vi "TargetArchsHasBin.vi"(8 "error in":errorcluster, 10 "MinorVersion":i32, 11 "MajorVersion":i32) -> (0 "error out":errorcluster, 3 "HasBinary":bool)   [LabVIEW 2020, in "OpenLvVision_OpenCv.lvlib" / "Cuda.lvlib"]
doc: "Check whether the module contains binary CUDA code for the given architecture"
uses:
  Cuda.lvlib
  OpenLvVision_OpenCv.lvlib
  <vilib>/Utility/error.llb/Error Cluster From Error Code.vi
  <vilib>/ErrorRing/Error Ring.xnode
  Dlls/OlvOpenCvWrapper.dll
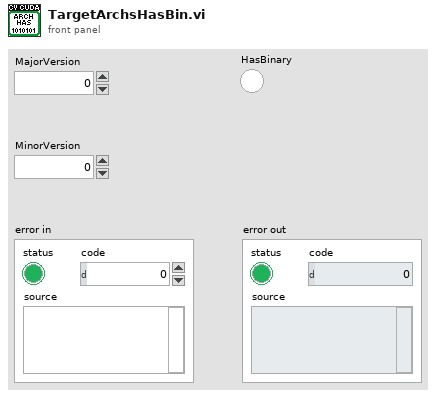
[diagram p1: front panel]
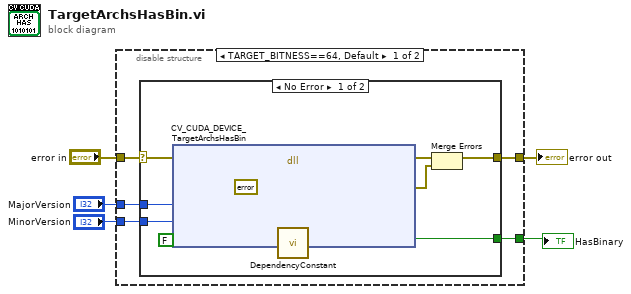
[diagram p0: block diagram]
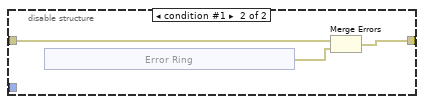
[diagram p3: hidden frame]
diagram:
  n1 = disable-structure shown="TARGET_BITNESS==64, Default" {
    disable-tunnel: "error in" -> [w9 w23]
    disable-tunnel: [w10 w22] -> w4
    disable-tunnel: "MajorVersion" -> [w8 _]
    disable-tunnel: "MinorVersion" -> [w7 _]
    disable-tunnel: [w6 _] -> w1
    frame condition #0 (active) {
      n2 = case shown="No Error" w9 {
        selector: w9 -> [w15 w20]
        tunnel: [w16 w20] -> w10
        tunnel: w8 -> [w14 _]
        tunnel: w7 -> [w13 _]
        tunnel: [w11 _] -> w6
        frame No Error {
          n3 = dll-call lib="C:/Users/lukas/Documents/OpenLvVision_OpenCv/SourceCode/LabView/OpenLvVision_OpenCv/Dlls/OlvOpenCvWrapper.dll" fn="CV_CUDA_DEVICE_TargetArchsHasBin"(error in=w15, "Error"=errorcluster {"status"=FALSE, "code"=0, "source"=""} ("error out"), "major"=w14, "minor"=w13, "result"=FALSE) -> (error out=w19:errorcluster, "Error"=w18:errorcluster, "result"=w11:bool)  [unwired: 5 in, 1 out]
          n4 = call "DependencyConstant.vi"() -> ()  [unwired: 12 in]
          n5 = Merge Errors(w19, w18) -> (w16:errorcluster)
        }
        frame Error {
        }
      }
    }
    frame condition #1 {
      n6 = xnode "Error Ring"() -> ("error out"=w21:errorcluster)
      n7 = Merge Errors(w23, w21) -> (w22:errorcluster)
    }
  }
  "error out" <- w4
  "HasBinary" <- w1
